vi "set Sweep Type.vi"(8 "error in (no error)":errorcluster, 10 "Sweep Mode":T1, 11 "Keysight 9020A in":refnum<class "Keysight 9020A.lvclass">) -> (0 "error out":errorcluster, 3 "Keysight 9020A out":refnum<class "Keysight 9020A.lvclass">)   [LabVIEW 2023, in "Spectrum Analyzer.lvlib" / "Keysight 9020A.lvclass"]
uses:
  Keysight 9020A.lvclass
  TYPE DEFINITION/TYPE Sweep Type Select.ctl
  Keysight 9020A.lvclass/Keysight 9020A.ctl
  Spectrum Analyzer.lvlib
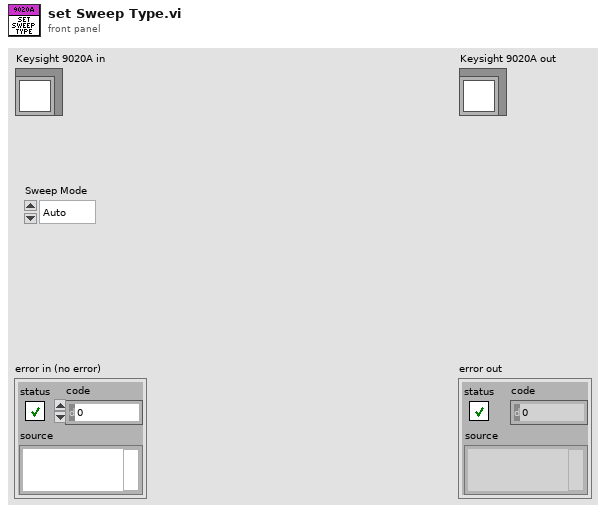
[diagram p1: front panel]
types:
  T1 = typedef "Spectrum Analyzer.lvlib/TYPE Sweep Type Select.ctl" = enum16{"Auto", "Sweep", "FFT"}
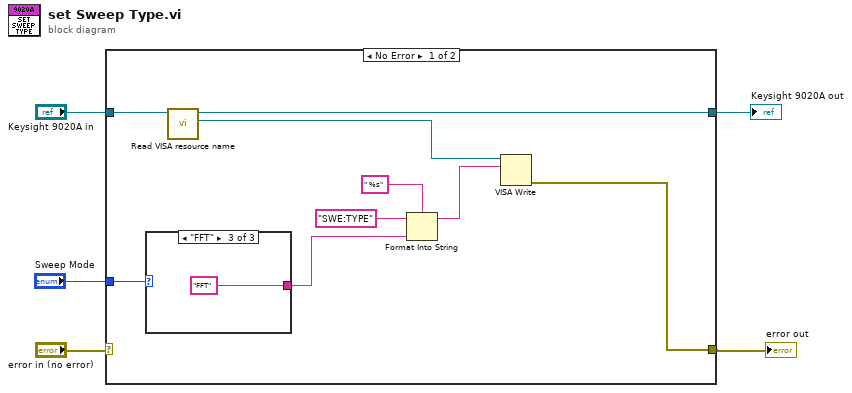
[diagram p0: block diagram]
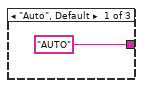
[diagram p2: hidden frame]
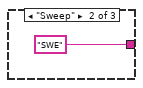
[diagram p3: hidden frame]
diagram:
  n1 = case shown="No Error" "error in (no error)" {
    selector: "error in (no error)" -> [_ w18]
    tunnel: "Keysight 9020A in" -> [w14 w19]
    tunnel: [w13 w19] -> w4
    tunnel: [w9 w18] -> w1
    tunnel: "Sweep Mode" -> [w8 _]
    frame No Error {
      n2 = case shown="\"FFT\"" w8 {
        tunnel: ["AUTO" "SWE" "FFT"] -> w7
        frame "Auto", Default {
        }
        frame "Sweep" {
        }
        frame "FFT" {
        }
      }
      n3 = call "Read VISA resource name.vi"("Keysight 9020A in"=w14) -> ("VISA resource name"=w6:refnum<visa-resource-name>, "Keysight 9020A out"=w13:refnum<class "Keysight 9020A.lvclass">)  [unwired: 8 in, 1 out]
      n4 = Format Into String(format string=" %s", initial string="SWE:TYPE", w7) -> (resulting string=w10:string)  [unwired: 1 in, 1 out]
      n5 = VISA Write(VISA resource name=w6, write buffer=w10) -> (error out=w9:errorcluster)  [unwired: 1 in, 2 out]
    }
    frame Error {
    }
  }
  "error out" <- w1
  "Keysight 9020A out" <- w4
